vi "Start Tick.vi"(8 "error in":errorcluster, 11 "Actor in":refnum<class "VTU Sim Rig.lvclass">) -> (0 "error out":errorcluster, 3 "Actor out":refnum<class "VTU Sim Rig.lvclass">)   [LabVIEW 2026, in "VTU Sim Rig.lvclass"]
doc: "Actor Core hook (series, before Call Parent). Starts a Time-Delayed Send Message of Tick Msg to the rig itself every 100 ms, repeat forever. The delivery notifier is left unwired: the AF helper stops itself when the actor's queue is destroyed on stop."
uses:
  VTU Sim Rig.lvclass
  Messages/Tick Msg/Tick Msg.lvclass
  <vilib>/ActorFramework/Actor/Actor.lvclass/Actor.ctl
  <vilib>/ActorFramework/Message Enqueuer/Message Enqueuer.lvclass/Message Enqueuer.ctl
  <vilib>/ActorFramework/Message Enqueuer/Init from Existing Queue.vi
  <vilib>/ActorFramework/Message Enqueuer/Message Enqueuer.lvclass
  <vilib>/ActorFramework/Actor/Actor.lvclass
  <vilib>/ActorFramework/Actor Framework.lvlib
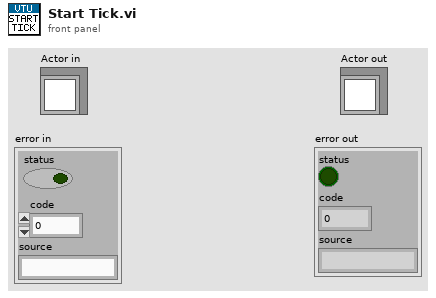
[diagram p1: front panel]
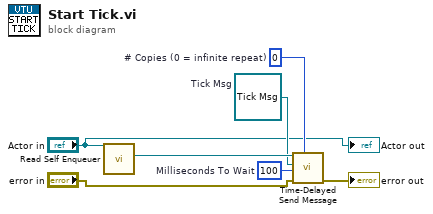
[diagram p0: block diagram]
diagram:
  w5 = u32 0  # # Copies (0 = infinite repeat)
  w4 = 100  # Milliseconds To Wait
  w3 = refnum<class "Tick Msg.lvclass"> refnum  # Tick Msg
  n1 = call <vilib>:"Read Self Enqueuer.vi"("Actor"="Actor in") -> ("Self Enqueuer"=w6:refnum<class "Message Enqueuer.lvclass">)  [unwired: 10 in]
  n2 = call <vilib>:"Time-Delayed Send Message.vi"("# Copies (0 = infinite repeat)"=w5, "error in (no error)"="error in", "Milliseconds To Wait"=w4, "Message"=w3, "Message Enqueuer"=w6) -> ("error out"=→"error out":errorcluster)  [unwired: 5 in, 1 out]
  "Actor out" <- "Actor in"
